vi "isProcedureCompatible.vi"(11 "Manual Test Data":string) -> (3 "Compatible":bool)   [LabVIEW 2026, in "dependencies.lvlib"]
uses:
  dependencies.lvlib
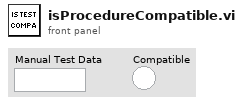
[diagram p1: front panel]
types:
  T1 = cluster{"Scope":string, "Setup":string, "Main":string, "Cleanup":string}
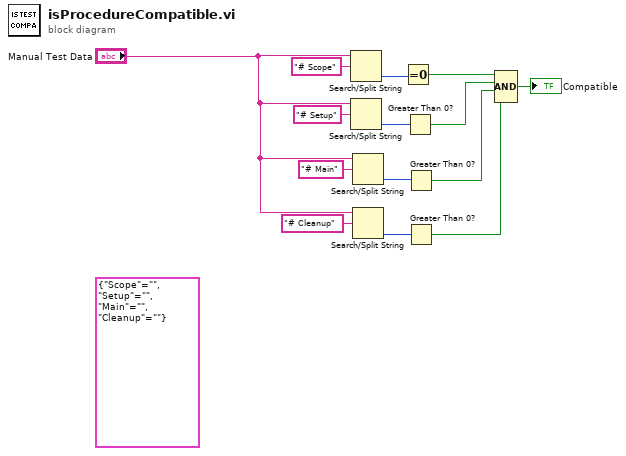
[diagram p0: block diagram]
diagram:
  (unwired) T1 {"Scope"="", "Setup"="", "Main"="", "Cleanup"=""}
  n1 = Search/Split String(string="Manual Test Data", search string/char (-)="# Scope") -> (offset of match=w10:i32)  [unwired: 1 in, 2 out]
  n2 = Search/Split String(string="Manual Test Data", search string/char (-)="# Setup") -> (offset of match=w9:i32)  [unwired: 1 in, 2 out]
  n3 = Search/Split String(string="Manual Test Data", search string/char (-)="# Main") -> (offset of match=w8:i32)  [unwired: 1 in, 2 out]
  n4 = Search/Split String(string="Manual Test Data", search string/char (-)="# Cleanup") -> (offset of match=w7:i32)  [unwired: 1 in, 2 out]
  n5 = Equal To 0?(x=w10) -> (x = 0?=w6:bool)
  n6 = Greater Than 0?(x=w9) -> (x > 0?=w3:bool)
  n7 = Greater Than 0?(x=w8) -> (x > 0?=w4:bool)
  n8 = Greater Than 0?(x=w7) -> (x > 0?=w5:bool)
  n9 = Compound Arithmetic op=AND(w6, w3, w4, w5) -> (→"Compatible":bool)
